vi "Load Motor Scale Parameter.vi"(8 "error in (no error)":errorcluster, 10 "Motor in":refnum<class "Motor.lvclass">, 11 "config file in":path) -> (0 "error out":errorcluster, 2 "Motor out":refnum<class "Motor.lvclass">, 3 "config file out":path)   [LabVIEW 2021]
uses:
  Motor/Motor.lvclass
  Motor/Motor.lvclass/Motor.ctl
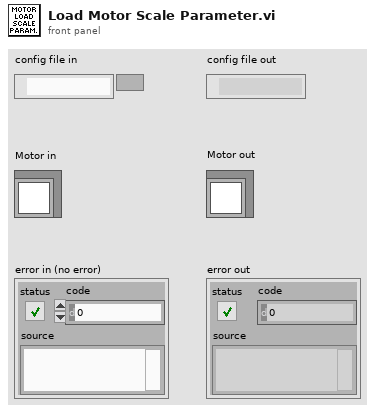
[diagram p1: front panel]
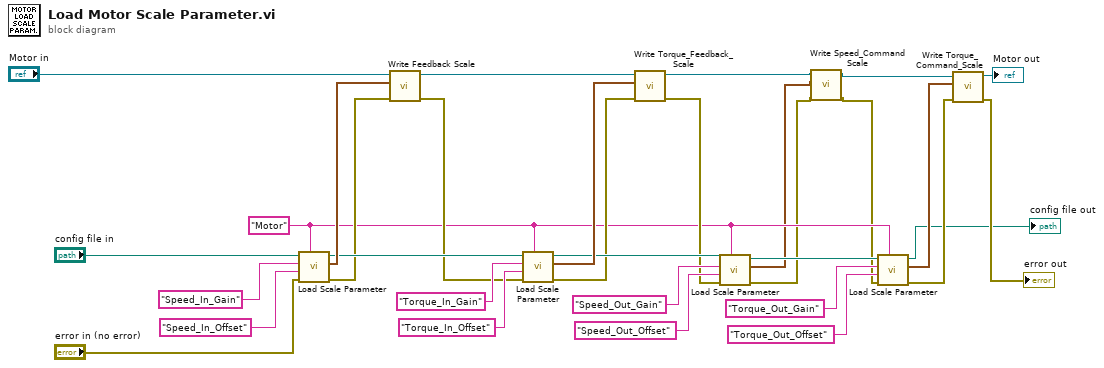
[diagram p0: block diagram]
diagram:
  w11 = "Motor" ("section")
  n1 = call "Load Scale Parameter.vi"("section"=w11, "error in (no error)"="error in (no error)", "Offset Key"="Speed_In_Offset", "Gain Key"="Speed_In_Gain", "config file in"="config file in") -> ("error out"=w18:errorcluster, "Scale Parameters"=w26:cluster{"Gain":dbl, "Offset":dbl}, "config file out"=w25:path)  [unwired: 4 in]
  n2 = call "Write Feedback Scale.vi"("error in (no error)"=w18, "Feedback Scale"=w26, "Motor in"="Motor in") -> ("error out"=w17:errorcluster, "Motor out"=w23:refnum<class "Motor.lvclass">)  [unwired: 7 in]
  n3 = call "Load Scale Parameter.vi"("section"=w11, "error in (no error)"=w17, "Offset Key"="Torque_In_Offset", "Gain Key"="Torque_In_Gain", "config file in"=w25) -> ("error out"=w16:errorcluster, "Scale Parameters"=w22:cluster{"Gain":dbl, "Offset":dbl}, "config file out"=w19:path)  [unwired: 4 in]
  n4 = call "Write Torque_Feedback_Scale.vi"("error in (no error)"=w16, "Torque_Feedback_Scale"=w22, "Motor in"=w23) -> ("error out"=w15:errorcluster, "Motor out"=w5:refnum<class "Motor.lvclass">)  [unwired: 7 in]
  n5 = call "Load Scale Parameter.vi"("section"=w11, "error in (no error)"=w15, "Offset Key"="Speed_Out_Offset", "Gain Key"="Speed_Out_Gain", "config file in"=w19) -> ("error out"=w2:errorcluster, "Scale Parameters"=w1:cluster{"Gain":dbl, "Offset":dbl}, "config file out"=w12:path)  [unwired: 4 in]
  n6 = call "Write Speed_Command Scale.vi"("error in (no error)"=w2, "Speed_Command Scale"=w1, "Motor in"=w5) -> ("error out"=w3:errorcluster, "Motor out"=w4:refnum<class "Motor.lvclass">)  [unwired: 7 in]
  n7 = call "Load Scale Parameter.vi"("section"=w11, "error in (no error)"=w3, "Offset Key"="Torque_Out_Offset", "Gain Key"="Torque_Out_Gain", "config file in"=w12) -> ("error out"=w9:errorcluster, "Scale Parameters"=w10:cluster{"Gain":dbl, "Offset":dbl}, "config file out"=→"config file out":path)  [unwired: 4 in]
  n8 = call "Write Torque_Command_Scale.vi"("error in (no error)"=w9, "Torque_Command_Scale"=w10, "Motor in"=w4) -> ("error out"=→"error out":errorcluster, "Motor out"=→"Motor out":refnum<class "Motor.lvclass">)  [unwired: 7 in]
